vi "DAC Run.vi"(8 "error in":errorcluster, 11 "DAC ADV in":refnum<class "DAC ADV.lvclass">) -> (0 "error out":errorcluster, 3 "DAC ADV out":refnum<class "DAC ADV.lvclass">)   [LabVIEW 2019, in "DAC.lvlib" / "DAC ADV.lvclass"]
uses:
  DAC ADV.lvclass
  C:/Users/wg/Documents/LV_Projects/test-stand/App/DAC/DAC.lvclass
  DAC.lvclass/DAC.ctl
  Results/Results Method.ctl
  Results/Water Tunnel Results/Water Tunnel Results.lvclass
  DAC ADV.lvclass/DAC ADV.ctl
  DAC.lvclass
  Results/Results.lvlib
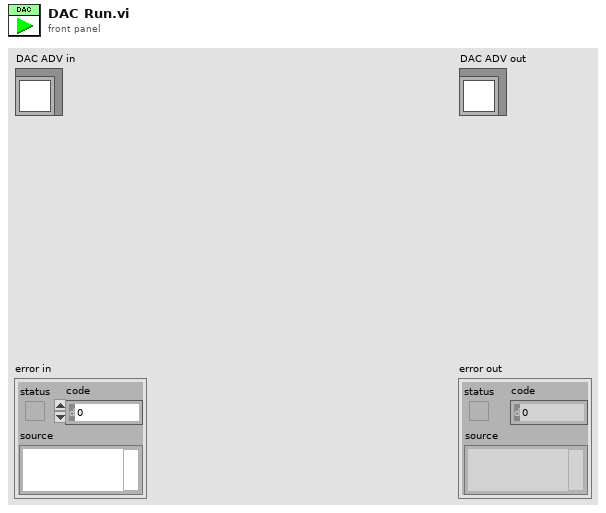
[diagram p1: front panel]
types:
  T1 = typedef "Results.lvlib/Results Method.ctl" = enum16{"Get", "Set"}
  T2 = cluster{"Vx":dbl, "Vy":dbl, "Vz":dbl, "Amplitude":dbl[], "Correlation":dbl[]}
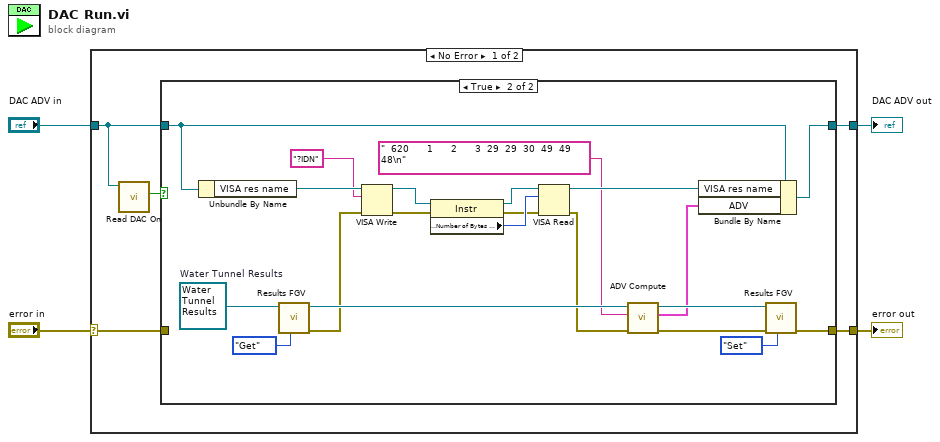
[diagram p0: block diagram]
diagram:
  n1 = case shown="No Error" "error in" {
    selector: "error in" -> [w7 w34]
    tunnel: [w6 w34] -> w2
    tunnel: [w8 w33] -> w1
    tunnel: "DAC ADV in" -> [w5 w33]
    frame No Error {
      n2 = call "Read DAC On.vi"("DAC in"=w5) -> ("DAC On"=w9:bool)  [unwired: 8 in, 2 out]
      n3 = case shown="True" w9 {
        tunnel: w5 -> [w11 w32]
        tunnel: [w11 w29] -> w8
        tunnel: w7 -> [w10 _]
        tunnel: [w10 w28] -> w6
        frame False {
        }
        frame True {
          w27 = refnum<class "Water Tunnel Results.lvclass"> refnum  # Water Tunnel Results
          n4 = Unbundle By Name(w32) -> ("VISA res name"=w16:refnum<visa-resource-name>)
          n5 = call-dynamic "Results FGV.vi"("Method"=Results_Method."Get", "Water Tunnel Results in"=w27) -> ("error out"=w14:errorcluster, "Water Tunnel  Results out"=w25:refnum<class "Water Tunnel Results.lvclass">)  [unwired: 8 in]
          n6 = VISA Write(VISA resource name=w16, write buffer="?IDN", error in (no error)=w14) -> (VISA resource name out=w13:refnum<visa-resource-name>, error out=w15:errorcluster)  [unwired: 1 out]
          n7 = property class="Instr"(reference=w13, error in=w15) -> (reference out=w19:refnum<visa-resource-name>, error out=w17:errorcluster, "Serial Settings:Number of Bytes at Serial Port"=w18:u32)
          n8 = VISA Read(VISA resource name=w19, byte count=w18, error in (no error)=w17) -> (VISA resource name out=w26:refnum<visa-resource-name>, error out=w23:errorcluster)  [unwired: 2 out]
          n9 = call "ADV Compute.vi"("error in"=w23, "ADV String"="  620      1      2      3  29  29  30  49  49  48\n", "Water Tunnel Results in"=w25) -> ("error out"=w22:errorcluster, "ADV"=w21:T2, "Water Tunnel Results out"=w24:refnum<class "Water Tunnel Results.lvclass">)  [unwired: 6 in]
          n10 = Bundle By Name(cluster=w32, "VISA res name"=w26, "ADV"=w21) -> (w29:refnum<class "DAC ADV.lvclass">)
          n11 = call-dynamic "Results FGV.vi"("Method"=Results_Method."Set", "error in"=w22, "Water Tunnel Results in"=w24) -> ("error out"=w28:errorcluster)  [unwired: 7 in, 1 out]
        }
      }
    }
    frame Error {
    }
  }
  "error out" <- w2
  "DAC ADV out" <- w1
